vi "CanWriterCansub GetCANStatus.vi"(6 "contextId":T1, 8 "error in":errorcluster, 9 "timeout (ms)":i32=-1, 10 "Request Data":T5, 11 "gRPC ID":T1) -> (0 "error out":errorcluster, 2 "Response Data":T2, 3 "gRPC ID out":T1)   [LabVIEW 2021, in "CanWriterCansub_client.lvlib"]
uses:
  CanWriterCansub_client.lvlib
  <vilib>/gRPC/LabVIEW gRPC Library/Shared/grpcId.ctl
  RPC Messages/cif_can_writer_cansub_GetCANStatusRequest.ctl
  RPC Messages/cif_can_writer_cansub_GetCANStatusResponse.ctl
  RPC Messages/cif_can_writer_cansub_CommState.ctl
  RPC Messages/cif_can_writer_cansub_LastError.ctl
  RPC Messages/cif_can_writer_cansub_GetCANStatusResponse_Flat.ctl
  14035477-4c25-4107-8ed5-d0c4ef420ce5.vi
  <vilib>/gRPC/LabVIEW gRPC Library/Shared/TranslateGrpcError.vi
  <vilib>/gRPC/LabVIEW gRPC Library/Shared/Wait On Occurrence.vi
  <vilib>/gRPC/LabVIEW gRPC Library/Shared/Is Feature Enabled.vi
  <vilib>/gRPC/LabVIEW gRPC Library/Server API/Server/Get Server DLL Path.vi
  <vilib>/Utility/error.llb/Error Cluster From Error Code.vi
  <vilib>/gRPC/LabVIEW gRPC Library/grpc-lvsupport-release.lvlib
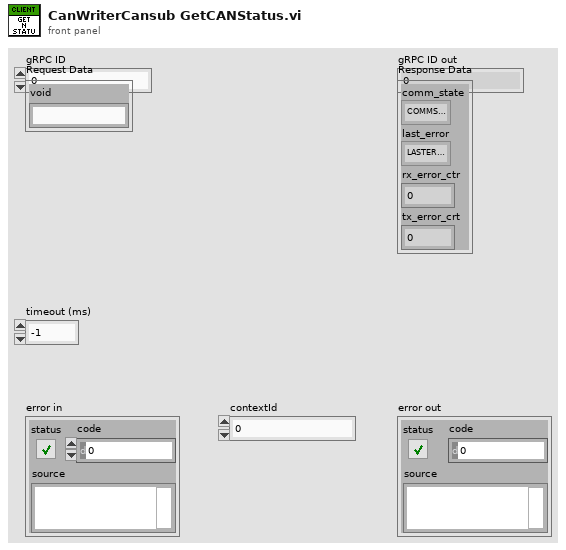
[diagram p1: front panel]
types:
  T1 = typedef "grpc-lvsupport-release.lvlib/grpcId.ctl" = u64
  T2 = typedef "CanWriterCansub_client.lvlib/cif_can_writer_cansub_GetCANStatusResponse.ctl" = cluster{"comm_state":T3, "last_error":T4, "rx_error_ctr":u32, "tx_error_crt":u32}
  T3 = typedef "CanWriterCansub_client.lvlib/cif_can_writer_cansub_CommState.ctl" = enum32{"COMMSTATE_ERROR_ACTIVE", "COMMSTATE_ERROR_PASSIVE", "COMMSTATE_BUS_OFF"}
  T4 = typedef "CanWriterCansub_client.lvlib/cif_can_writer_cansub_LastError.ctl" = enum32{"LASTERROR_NONE", "LASTERROR_STUFF", "LASTERROR_FORM", "LASTERROR_ACK", "LASTERROR_BIT1", "LASTERROR_BIT0", "LASTERROR_CRC", "LASTERROR_UNKNOWN"}
  T5 = typedef "CanWriterCansub_client.lvlib/cif_can_writer_cansub_GetCANStatusRequest.ctl" = cluster{"void":string}
  T6 = typedef "CanWriterCansub_client.lvlib/cif_can_writer_cansub_GetCANStatusResponse_Flat.ctl" = cluster{"comm_state":T3, "last_error":T4, "rx_error_ctr":u32, "tx_error_crt":u32}
  T7 = typedef "CanWriterCansub_client.lvlib/cif_can_writer_cansub_GetCANStatusRequest_Flat.ctl" = cluster{"void":string}
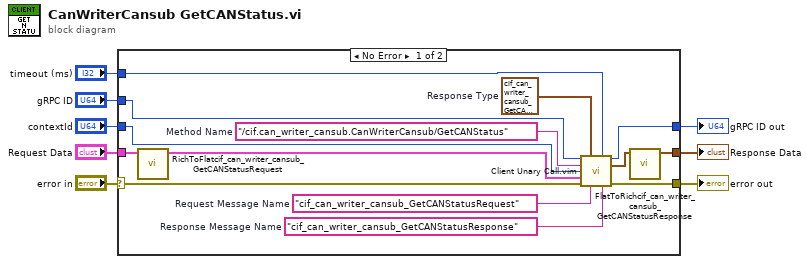
[diagram p0: block diagram]
diagram:
  n1 = case shown="No Error" "error in" {
    selector: "error in" -> [w18 w23]
    tunnel: [w17 w23] -> w7
    tunnel: "gRPC ID" -> [w16 w24]
    tunnel: [w15 w24] -> w5
    tunnel: "Request Data" -> [w12 _]
    tunnel: [w9 _] -> w3
    tunnel: "timeout (ms)" -> [w14 _]
    tunnel: "contextId" -> [w13 _]
    frame No Error {
      w19 = "cif_can_writer_cansub_GetCANStatusResponse"  # Response Message Name
      w20 = "cif_can_writer_cansub_GetCANStatusRequest"  # Request Message Name
      w21 = T6 {"comm_state"=enum."COMMSTATE_ERROR_ACTIVE", "last_error"=enum."LASTERROR_NONE", "rx_error_ctr"=0, "tx_error_crt"=0}  # Response Type
      w22 = "/cif.can_writer_cansub.CanWriterCansub/GetCANStatus"  # Method Name
      n2 = call "RichToFlatcif_can_writer_cansub_GetCANStatusRequest.vi"("InputCluster"=w12) -> ("OutputCluster"=w11:T7)  [unwired: 10 in]
      n3 = call "Client Unary Call.vim"("ClientID in"=w16, "Response Type"=w21, "timeout (ms)"=w14, "Method Name"=w22, "contextId"=w13, "Request Data"=w11, "error in"=w18, "Request Message Name"=w20, "Response Message Name"=w19) -> ("ClientID out"=w15:T1, "Response Data"=w10:T6, "error out"=w17:errorcluster)  [unwired: 4 in]
      n4 = call "FlatToRichcif_can_writer_cansub_GetCANStatusResponse.vi"("InputCluster"=w10) -> ("OutputCluster"=w9:T2)  [unwired: 10 in]
    }
    frame Error {
    }
  }
  "error out" <- w7
  "gRPC ID out" <- w5
  "Response Data" <- w3
